vi "Reset Switch Power Reset .vi"() -> (0 "error out":errorcluster, 2 "Result":string, 3 "Result":bool)   [LabVIEW 2021]
uses:
  10054_Control Folder/Support/Relay_no.ctl
panel:
  out "status":bool
  in  "error in (no error)":errorcluster
  out ".not. x?":bool
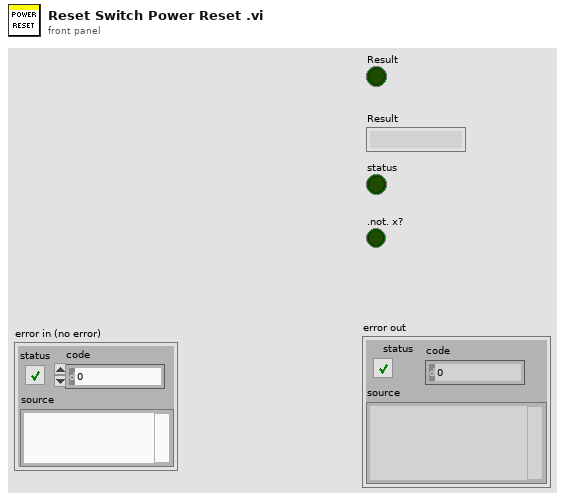
[diagram p1: front panel]
types:
  T1 = typedef "Relay_no.ctl" = enum16{"Init", "write&Read", "PCB Serial Write & Read", "PCB Write SSD & Password", "Read Wifi state", "Reset", "Close"}
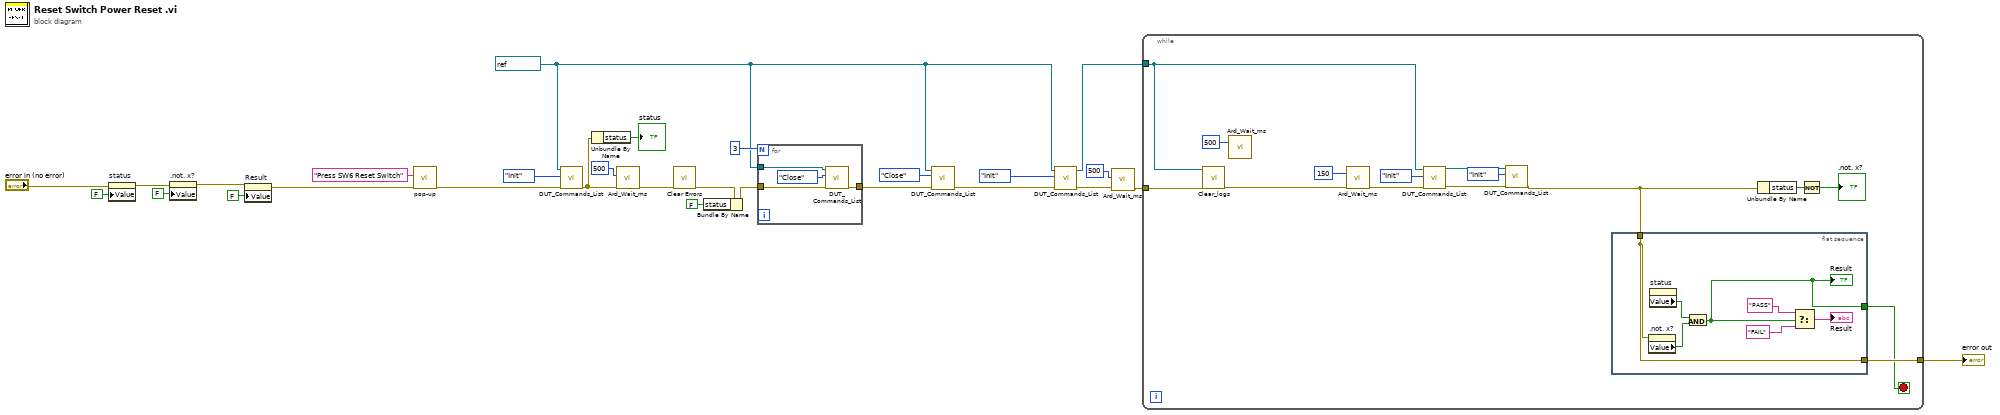
[diagram p0: block diagram]
diagram:
  w10 = refnum<visa-resource-name> "COM3" ("Resource In")
  n1 = property on="status" class="Bool (strict)"(error in="error in (no error)", "Value"=FALSE ("status")) -> (error out=w9:errorcluster)  [unwired: 1 in, 1 out]
  n2 = property on=".not. x?" class="Bool (strict)"(error in=w9, "Value"=FALSE (".not. x?")) -> (error out=w8:errorcluster)  [unwired: 1 in, 1 out]
  n3 = property on="Result" class="Bool (strict)"(error in=w8, "Value"=FALSE ("Result")) -> (error out=w3:errorcluster)  [unwired: 1 in, 1 out]
  n4 = call "pop-up.vi"("error in"=w3, "input string"="Press SW6 Reset Switch") -> ("error out"=w2:errorcluster)  [unwired: 7 in, 2 out]
  n5 = call "DUT_Commands_List.vi"("error in"=w2, "Operation"=Relay_no."Init", "Resource In"=w10) -> ("error out"=w24:errorcluster)  [unwired: 6 in, 2 out]
  n6 = Unbundle By Name(w24) -> ("status"=→"status":bool)
  n7 = call "Ard_Wait_ms.vi"("error in"=w24, "millisec"=u32 500) -> ("error in 2"=w23:errorcluster)  [unwired: 9 in]
  n8 = call <vilib>:"Clear Errors.vi"("error in (no error)"=w23) -> ("error out"=w21:errorcluster)  [unwired: 5 in, 1 out]
  n9 = Bundle By Name(cluster=w21, "status"=FALSE) -> (w19:errorcluster)
  n10 = for {
    N: 3 -> [_]
    tunnel: w10 -> [w29]
    tunnel: w19 -> [w31]
    tunnel: [w30] -> w17
    n11 = call "DUT_Commands_List.vi"("error in"=w31, "Operation"=Relay_no."Close", "Resource In"=w29) -> ("error out"=w30:errorcluster)  [unwired: 6 in, 2 out]
  }
  n12 = call "DUT_Commands_List.vi"("error in"=w17, "Operation"=Relay_no."Close", "Resource In"=w10) -> ("error out"=w16:errorcluster)  [unwired: 6 in, 2 out]
  n13 = call "DUT_Commands_List.vi"("error in"=w16, "Operation"=Relay_no."Init", "Resource In"=w10) -> ("error out"=w12:errorcluster, "Resource out"=w4:refnum<visa-resource-name>)  [unwired: 6 in, 1 out]
  n14 = call "Ard_Wait_ms.vi"("error in"=w12, "millisec"=u32 500) -> ("error in 2"=w11:errorcluster)  [unwired: 9 in]
  n15 = while {
    tunnel: [w41] -> w28
    tunnel: w11 -> [w38]
    tunnel: w4 -> [w39]
    stop <- w40 stop-if-true
    n16 = call "Clear_logs.vi"("error in (no error)"=w38, "VISA resource name"=w39) -> ("error out"=w45:errorcluster)  [unwired: 4 in, 3 out]
    n17 = call "Ard_Wait_ms.vi"("millisec"=u32 500) -> ()  [unwired: 10 in, 1 out]
    n18 = call "Ard_Wait_ms.vi"("error in"=w45, "millisec"=u32 150) -> ("error in 2"=w46:errorcluster)  [unwired: 9 in]
    n19 = call "DUT_Commands_List.vi"("error in"=w46, "Operation"=Relay_no."Init", "Resource In"=w39) -> ("error out"=w35:errorcluster, "Resource out"=w34:refnum<visa-resource-name>)  [unwired: 6 in, 1 out]
    n20 = call "DUT_Commands_List.vi"("error in"=w35, "Operation"=Relay_no."Init", "Resource In"=w34) -> ("error out"=w36:errorcluster)  [unwired: 6 in, 2 out]
    n21 = flat-sequence {
      tunnel: w36 -> [w50]
      tunnel: [w50] -> w41
      tunnel: [w49] -> w40
      frame #0 {
        n22 = property on=".not. x?" class="Bool (strict)"(error in=w50) -> ("Value"=w54:bool)  [unwired: 1 in, 2 out]
        n23 = property on="status" class="Bool (strict)"() -> ("Value"=w48:bool)  [unwired: 2 in, 2 out]
        n24 = And(x=w48, y=w54) -> (x .and. y?=w49:bool)
        "Result" <- w49
        n25 = Select(t="PASS", s=w49, f="FAIL") -> (s? t:f=→"Result":string)
      }
    }
    n26 = Unbundle By Name(w36) -> ("status"=w43:bool)
    n27 = Not(x=w43) -> (.not. x?=→".not. x?":bool)
  }
  "error out" <- w28
